vi "Choose Protocol Version.vi"(8 "error in":errorcluster, 11 "requested version":string) -> (0 "error out":errorcluster, 3 "protocol version":string)   [LabVIEW 2020, in "MCP Server.lvlib"]
doc: "Version negotiation of initialize.\n\nrequested version is the protocolVersion of the request as JSON text, for example \"2025-03-26\" with the quotes (empty if the request has none). If it is one of the versions in Supported Protocol Versions.vi, protocol version is that version. Otherwise it is the first entry of that list, the newest version this server supports.\n\nprotocol version is JSON text, ready for Set Item."
uses:
  MCP Server.lvlib
  141d4b81-f906-4748-8f18-4513d744ca10.vi
  45ea51fe-ed7e-4d0e-a415-fc1fb5b7f54b.vi
  <vilib>/JDP Science/JSONtext/JSON text to Variant.vi
  <vilib>/JDP Science/JSONtext/Variant to JSON Text.vi
  <vilib>/JDP Science/JSONtext/LVClass Serializer/JSONtext LVClass Serializer.lvclass
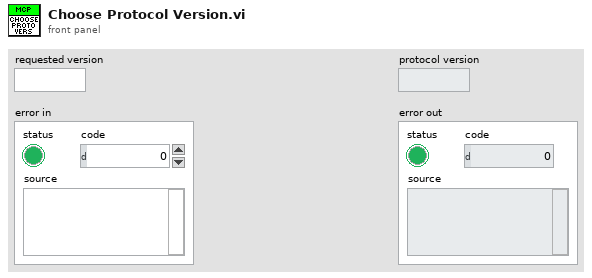
[diagram p1: front panel]
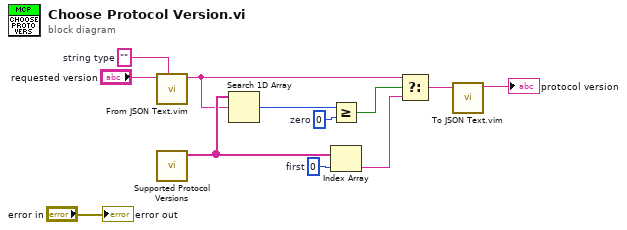
[diagram p0: block diagram]
diagram:
  w7 = 0  # first
  w9 = 0  # zero
  w11 = ""  # string type
  n1 = call "From JSON Text.vim"("Data Type and Default Value"=w11, "JSON"="requested version") -> ("Data out"=w6:string)  [unwired: 8 in, 1 out]
  n2 = call "Supported Protocol Versions.vi"() -> ("supported versions"=w8:string[])  [unwired: 11 in]
  n3 = Search 1D Array(1D array=w8, element=w6) -> (index of element=w10:i32)  [unwired: 1 in]
  n4 = Greater Or Equal?(x=w10, y=w9) -> (x >= y?=w5:bool)
  n5 = Index Array(array=w8, index=w7) -> (element=w4:string)
  n6 = Select(t=w6, s=w5, f=w4) -> (s? t:f=w3:string)
  n7 = call "To JSON Text.vim"("Anything"=w3) -> ("<JSON>"=→"protocol version":string)  [unwired: 9 in, 1 out]
  "error out" <- "error in"
